vi "Voltmeter read value.vi"(3 "error in":errorcluster, 5 "Voltmeter VISA in":refnum<visa-resource-name>) -> (0 "error out":errorcluster, 1 "Value":dbl format="%#_15p", 2 "Voltmeter VISA":refnum<visa-resource-name>)   [LabVIEW 2011]
doc: "Reads a value from the HP/Agilent 3458 multimeter."
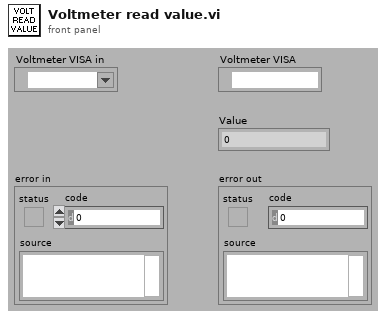
[diagram p1: front panel]
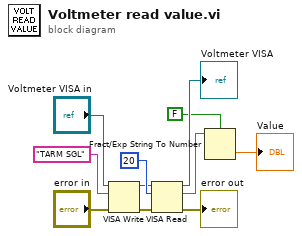
[diagram p0: block diagram]
diagram:
  n1 = VISA Write(VISA resource name="Voltmeter VISA in", write buffer="TARM SGL", error in (no error)="error in") -> (VISA resource name out=w3:refnum<visa-resource-name>, error out=w4:errorcluster)  [unwired: 1 out]
  n2 = VISA Read(VISA resource name=w3, byte count=u32 20, error in (no error)=w4) -> (VISA resource name out=→"Voltmeter VISA":refnum<visa-resource-name>, read buffer=w5:string, error out=→"error out":errorcluster)  [unwired: 1 out]
  n3 = Fract/Exp String To Number(use system decimal point (T)=FALSE, string=w5) -> (number=→"Value":dbl)  [unwired: 2 in, 1 out]
